vi "properties.to_json.vi"(8 "error in":errorcluster, 10 "properties":T1) -> (0 "error out":errorcluster, 2 "json":string)   [LabVIEW 2020, in "type.lvclass"]
uses:
  type.lvclass
  properties.ctl
  property.ctl
  property value.ctl
  89e06e07-596b-4f08-8f01-ad3ba62158ca.vi
  <vilib>/JDP Science/JSONtext/Variant to JSON Text.vi
  <vilib>/JDP Science/JSONtext/LVClass Serializer/JSONtext LVClass Serializer.lvclass
  type.lvclass/type.ctl
  <vilib>/JDP Science/JSONtext/JSONtext.lvlib
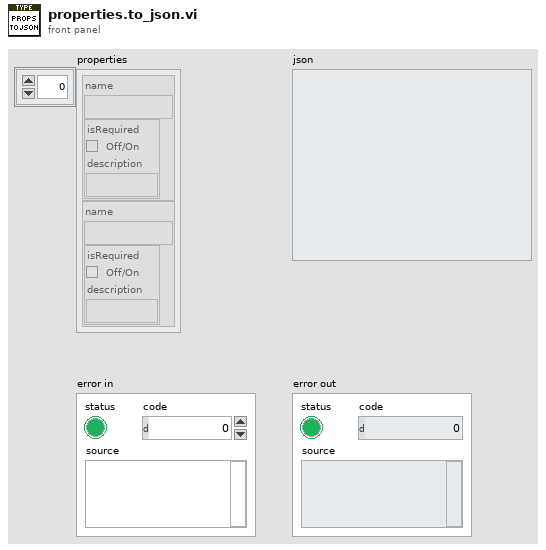
[diagram p1: front panel]
types:
  T1 = typedef "type.lvclass/properties.ctl" = T2[]
  T2 = typedef "type.lvclass/property.ctl" = cluster{"name":string, "value":T3}
  T3 = typedef "type.lvclass/property value.ctl" = cluster{"isRequired":bool, "description":string}
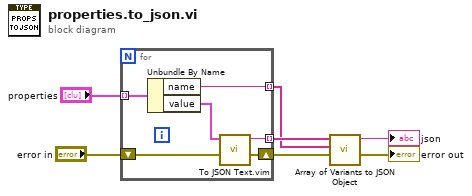
[diagram p0: block diagram]
diagram:
  n1 = for {
    tunnel: "properties" -> [w13] mode=indexing
    tunnel: [w11] -> w6 mode=indexing
    tunnel: [w10] -> w5 mode=indexing
    shift-right: [w9] -> w4
    shift-left: "error in" -> [w8]
    n2 = Unbundle By Name(w13) -> ("name"=w10:string, "value"=w12:T3)
    n3 = call "To JSON Text.vim"("error in (no error)"=w8, "Anything"=w12) -> ("error out"=w9:errorcluster, "<JSON>"=w11:string)  [unwired: 8 in]
  }
  n4 = call <vilib>:"Array of Variants to JSON Object.vi"("error in (no error)"=w4, "Names"=w5, "Array"=w6) -> ("error out"=→"error out":errorcluster, "<JSON>"=→"json":string)  [unwired: 7 in]
